vi "Initialize.vi"(8 "error in":errorcluster, 11 "Plugin in":refnum<class "Modbus.lvclass">) -> (0 "error out":errorcluster, 3 "Plugin out":refnum<class "Modbus.lvclass">)   [LabVIEW 2026, in "Modbus.lvlib" / "Modbus.lvclass"]
uses:
  Modbus.lvclass
  <vilib>/FlexLogger/SDK/PluginSDK.lvlibp/PEFClasses/SDK/Plugin/Plugin.lvclass
  C:/Program Files/National Instruments/LabVIEW 2026/vi.lib/FlexLogger/SDK/PluginSDK.lvlibp/PEFClasses/SDK/Plugin/Plugin.lvclass
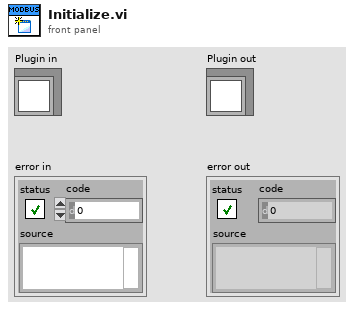
[diagram p1: front panel]
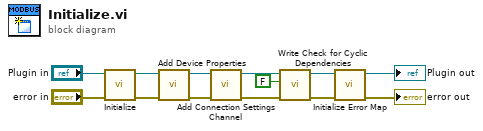
[diagram p0: block diagram]
diagram:
  n1 = call-parent "Initialize.vi"("error in (no error)"="error in", "Plugin in"="Plugin in") -> ("error out"=w8:errorcluster, "Plugin out"=w11:refnum<class "Modbus.lvclass">)  [unwired: 8 in]
  n2 = call "Add Device Properties.vi"("error in (no error)"=w8, "Modbus in"=w11) -> ("error out"=w5:errorcluster, "Modbus out"=w6:refnum<class "Modbus.lvclass">)  [unwired: 8 in]
  n3 = call "Add Connection Settings Channel.vi"("error in (no error)"=w5, "Modbus in"=w6) -> ("error out"=w10:errorcluster, "Modbus out"=w1:refnum<class "Modbus.lvclass">)  [unwired: 8 in]
  n4 = call <vilib>:"Write Check for Cyclic Dependencies.vi"("error in (no error)"=w10, "Check for Cyclic Dependencies?"=FALSE, "Plugin in"=w1) -> ("error out"=w7:errorcluster, "Plugin out"=w3:refnum<class "Modbus.lvclass">)  [unwired: 7 in]
  n5 = call "Initialize Error Map.vi"("error in (no error)"=w7, "Modbus in"=w3) -> ("error out"=→"error out":errorcluster, "Modbus out"=→"Plugin out":refnum<class "Modbus.lvclass">)  [unwired: 8 in]
